vi "NR check RB Status.vi"(8 "error in (no error)":errorcluster caption="에러 입력(에러 없음)", 9 "RB Offset":i32, 10 "RB Size":i32, 11 "Instrument Manager 입력":refnum<class "Instrument Manager.lvclass">) -> (0 "error out":errorcluster caption="에러 출력", 2 "Success?":bool, 3 "Instrument Manager 출력":refnum<class "Instrument Manager.lvclass">)   [LabVIEW 2023, in "Instrument Manager.lvclass"]
uses:
  Instrument Manager.lvclass
  Instrument Manager.lvclass/Instrument Manager.ctl
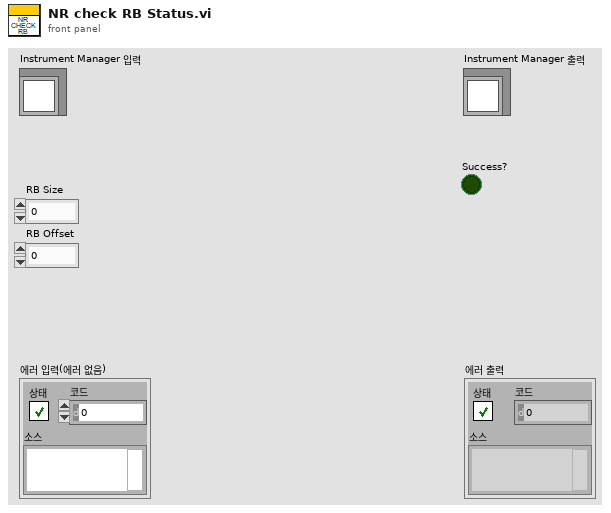
[diagram p1: front panel]
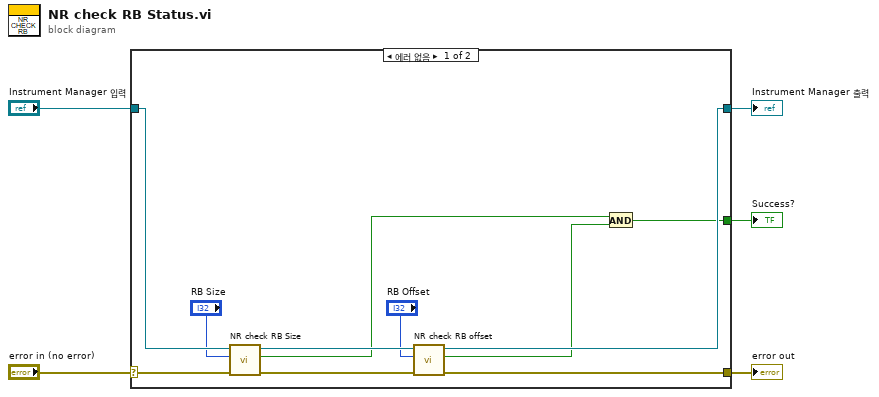
[diagram p0: block diagram]
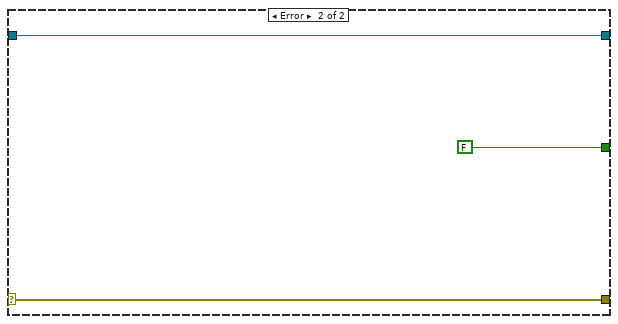
[diagram p2: hidden frame]
diagram:
  n1 = case shown="에러 없음" "error in (no error)" {
    selector: "error in (no error)" -> [w16 w19]
    tunnel: [w14 w19] -> w4
    tunnel: [w11 w18] -> w2
    tunnel: "Instrument Manager 입력" -> [w12 w18]
    tunnel: [w8 FALSE] -> w1
    frame No Error {
      n2 = call "NR check RB Size.vi"("error in (no error)"=w16, "RB Value (0~273)"="RB Size", "Instrument Manager 입력"=w12) -> ("error out"=w15:errorcluster, "Success?"=w10:bool, "Instrument Manager 출력"=w13:refnum<class "Instrument Manager.lvclass">)  [unwired: 6 in]
      n3 = call "NR check RB offset.vi"("error in (no error)"=w15, "RB Value (0~273)"="RB Offset", "Instrument Manager 입력"=w13) -> ("error out"=w14:errorcluster, "Success?"=w9:bool, "Instrument Manager 출력"=w11:refnum<class "Instrument Manager.lvclass">)  [unwired: 6 in]
      n4 = And(x=w10, y=w9) -> (x .and. y?=w8:bool)
    }
    frame Error {
    }
  }
  "error out" <- w4
  "Instrument Manager 출력" <- w2
  "Success?" <- w1
